vi "Add Server Certificate Paths.vi"(10 "Server Connection Configuration In":T1) -> (2 "Server Connection Configuration Out":T1)   [LabVIEW 2014, in "OPC UA Client Tests.lvlib"]
doc: "Add Certificate paths to Server configuration"
uses:
  OPC UA Client Tests.lvlib
  Server Connection Configuration.ctl
  <vilib>/OPCUA/server/subVI/supported security policies.ctl
  <vilib>/OPCUA/NI OPC UA Utility.lvlib
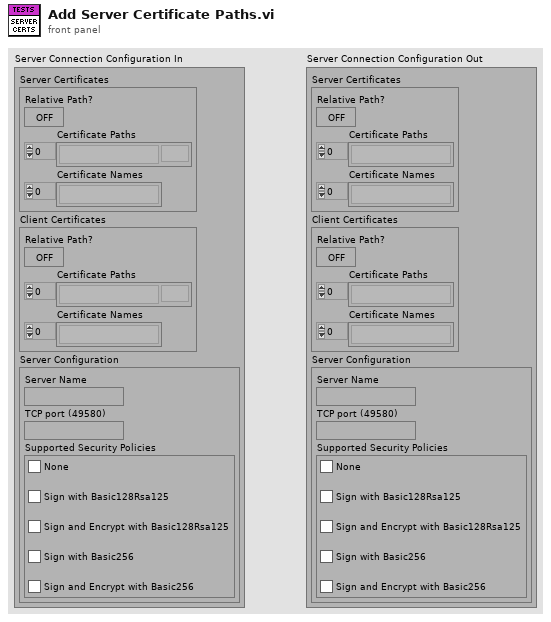
[diagram p1: front panel]
types:
  T1 = typedef "OPC UA Client Tests.lvlib/Server Connection Configuration.ctl" = cluster{"Server Certificates":cluster{"Relative Path?":bool, "Certificate Paths":path[], "Certificate Names":string[]}, "Client Certificates":cluster{"Relative Path?":bool, "Certificate Paths":path[], "Certificate Names":string[]}, "Server Configuration":cluster{"Server Name":string, "TCP port (49580)":string, "Supported Security Policies":T2}}
  T2 = typedef "supported security policies.ctl" = cluster{"None":bool, "Sign with Basic128Rsa125":bool, "Sign and Encrypt with Basic128Rsa125":bool, "Sign with Basic256":bool, "Sign and Encrypt with Basic256":bool}
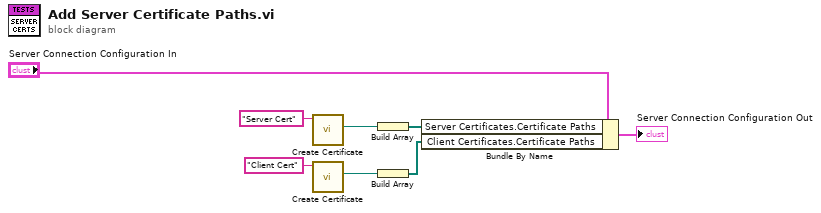
[diagram p0: block diagram]
diagram:
  n1 = call <vilib>:"Create Certificate.vi"("certificate name in"="Server Cert") -> ("certificate path"=w2:path)  [unwired: 7 in, 3 out]
  n2 = call <vilib>:"Create Certificate.vi"("certificate name in"="Client Cert") -> ("certificate path"=w1:path)  [unwired: 7 in, 3 out]
  n3 = Build Array(w2) -> (w7:path[])
  n4 = Build Array(w1) -> (w8:path[])
  n5 = Bundle By Name(cluster="Server Connection Configuration In", "Server Certificates.Certificate Paths"=w7, "Client Certificates.Certificate Paths"=w8) -> (→"Server Connection Configuration Out":T1)
